vi "SA mark Next Peak.vi"(8 "error in (no error)":errorcluster caption="에러 입력(에러 없음)", 10 "Marker Index":i32, 11 "Instrument Manager 입력":refnum<class "Instrument Manager.lvclass">) -> (0 "error out":errorcluster caption="에러 출력", 2 "Amplitude":dbl, 3 "Instrument Manager 출력":refnum<class "Instrument Manager.lvclass">)   [LabVIEW 2023, in "Instrument Manager.lvclass"]
uses:
  Instrument Manager.lvclass
  Module/Spectrum Analyzer/TYPE DEFINITION/TYPE Marker Control Mode.ctl
  Instrument Manager.lvclass/Instrument Manager.ctl
  Module/Spectrum Analyzer/Interface_Spectrum/Interface_Spectrum.lvclass
  Module/Spectrum Analyzer/Spectrum Analyzer.lvlib
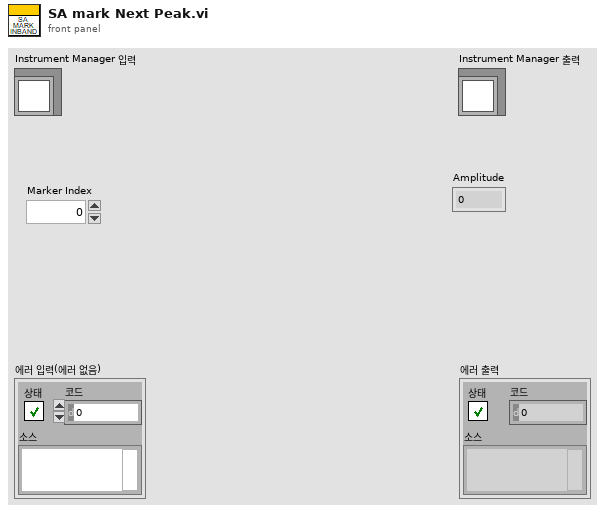
[diagram p1: front panel]
types:
  T1 = typedef "Spectrum Analyzer.lvlib/TYPE Marker Control Mode.ctl" = enum16{"Normal", "Delta", "Off"}
  T2 = cluster{"Anritsu Call Box":refnum<class "Anritsu Call Box.lvclass">, "Spectrum Analyzer":refnum<class "Interface_Spectrum.lvclass">, "RF Switch Box":refnum<class "RF Filter Box.lvclass">, "Turn Table":refnum<class "Interface - Turn Table.lvclass">, "Mast":refnum<class "Interface - Mast.lvclass">, "3D Controller":refnum<class "Interface_3D Controller.lvclass">}
  T3 = typedef "Spectrum Analyzer.lvlib/TYPE Marker Value.ctl" = cluster{"X-axis":dbl, "Y-axis":dbl}
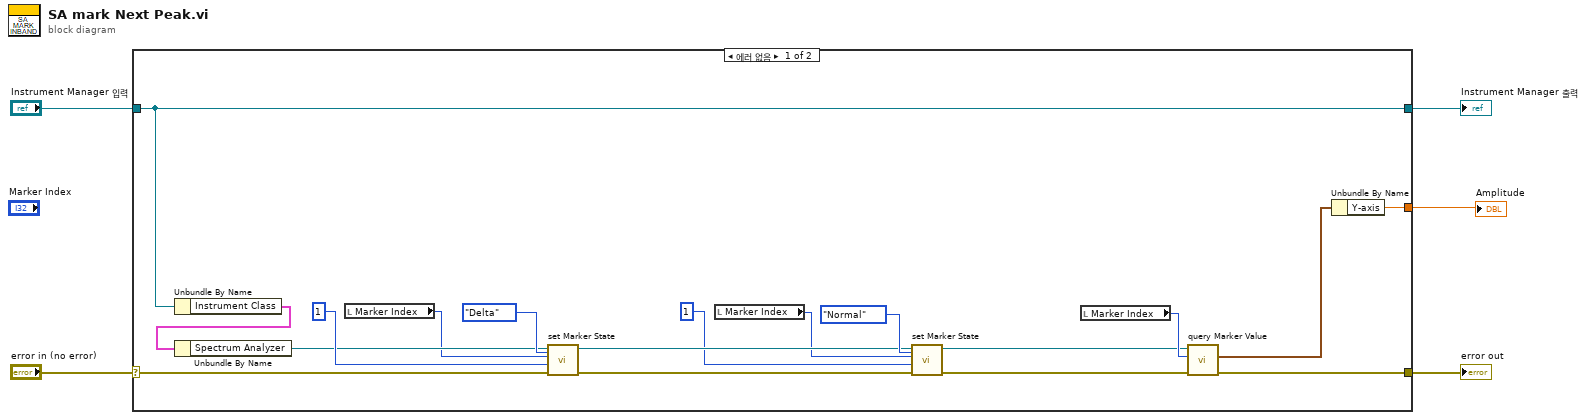
[diagram p0: block diagram]
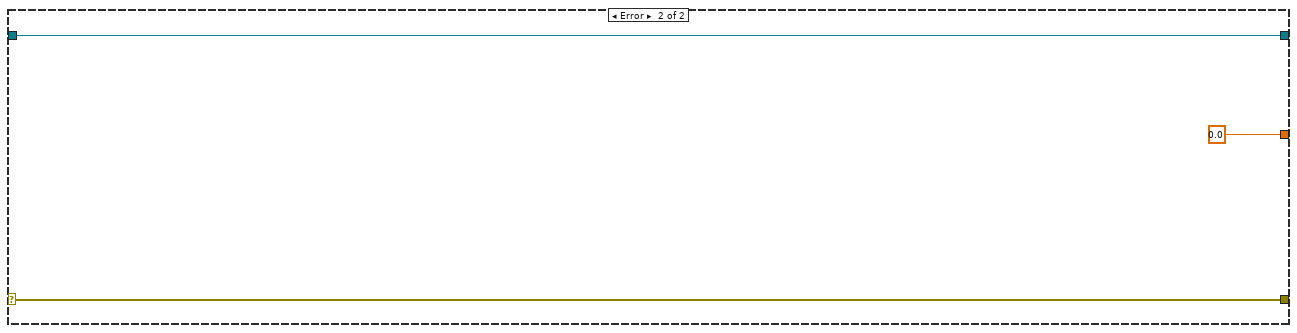
[diagram p2: hidden frame]
diagram:
  n1 = case shown="에러 없음" "error in (no error)" {
    selector: "error in (no error)" -> [w18 w26]
    tunnel: [w15 w26] -> w4
    tunnel: [w23 w25] -> w2
    tunnel: "Instrument Manager 입력" -> [w23 w25]
    tunnel: [w13 0.0 ("Y-axis")] -> w1
    frame No Error {
      n2 = Unbundle By Name(w23) -> ("Instrument Class"=w22:T2)
      n3 = Unbundle By Name(w22) -> ("Spectrum Analyzer"=w19:refnum<class "Interface_Spectrum.lvclass">)
      n4 = local read "Marker Index"() -> (w17:i32)
      n5 = call-dynamic "set Marker State.vi"("Marker Mode"=TYPE_Marker_Control_Mode."Delta", "error in (no error)"=w18, "trace index"=1, "Marker Index"=w17, "Interface_Spectrum in"=w19) -> ("error out"=w9:errorcluster, "Interface_Spectrum out"=w11:refnum<class "Interface_Spectrum.lvclass">)  [unwired: 5 in]
      n6 = local read "Marker Index"() -> (w7:i32)
      n7 = call-dynamic "set Marker State.vi"("Marker Mode"=TYPE_Marker_Control_Mode."Normal", "error in (no error)"=w9, "trace index"=1, "Marker Index"=w7, "Interface_Spectrum in"=w11) -> ("error out"=w8:errorcluster, "Interface_Spectrum out"=w10:refnum<class "Interface_Spectrum.lvclass">)  [unwired: 5 in]
      n8 = local read "Marker Index"() -> (w16:i32)
      n9 = call-dynamic "query Marker Value.vi"("error in (no error)"=w8, "Marker Index"=w16, "Interface_Spectrum in"=w10) -> ("error out"=w15:errorcluster, "Marker Value"=w14:T3)  [unwired: 6 in, 1 out]
      n10 = Unbundle By Name(w14) -> ("Y-axis"=w13:dbl)
    }
    frame Error {
    }
  }
  "error out" <- w4
  "Instrument Manager 출력" <- w2
  "Amplitude" <- w1
